vi "Tag.vi"(0 "obj in":refnum<class "Temp Sensor.lvclass">) -> (1 "tag":string)   [LabVIEW 2026, in "Temp Sensor.lvclass"]
doc: "Round15 P15: Temp Sensor's override of Sensor:Tag. Same shape; only the returned string differs, so a dispatched call reveals which implementation ran."
uses:
  Temp Sensor.lvclass
  Temp Sensor.lvclass/Temp Sensor.ctl
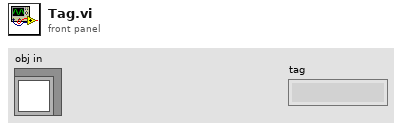
[diagram p1: front panel]
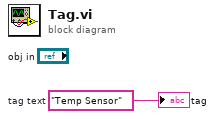
[diagram p0: block diagram]
diagram:
  w1 = "Temp Sensor"  # tag text
  "tag" <- w1
